vi "ADC_Config_Page.vi"() -> ()   [LabVIEW 2026, in "Core.lvlib"]
uses:
  Core.lvlib
  INL_DNL_Config_Page.vi
  TypeDefs/Enum_ADC_Tests.ctl
panel:
  in  "ADC Device Test":T1
  # "ADC Config Page"
  # "Instrument Specifications"
  # "Measurement Specifications"
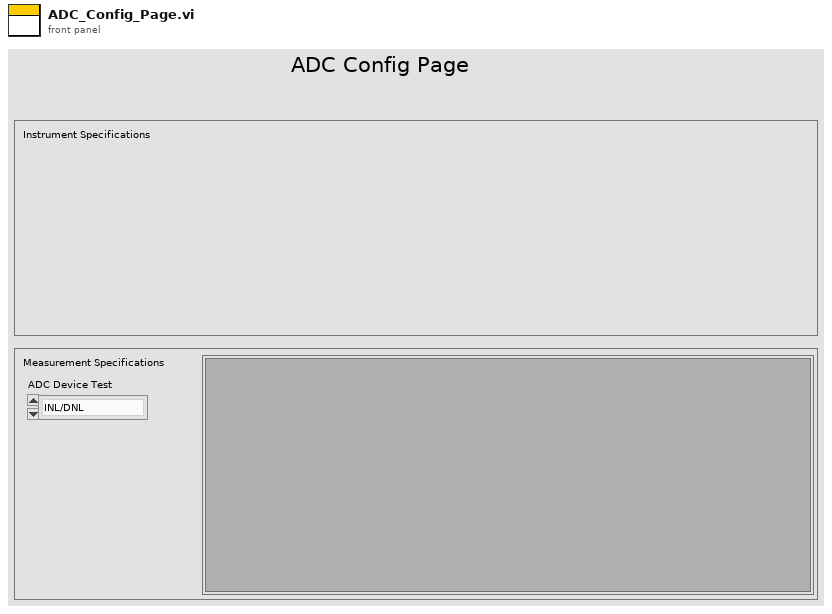
[diagram p1: front panel]
types:
  T1 = typedef "Core.lvlib/Enum_ADC_Tests.ctl" = enum16{"INL/DNL"}
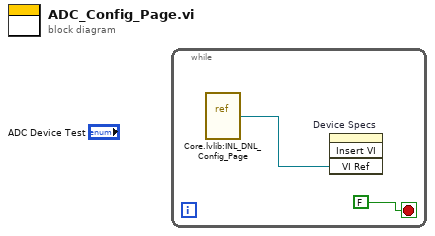
[diagram p0: block diagram]
diagram:
  n1 = while {
    stop <- FALSE stop-if-true
    n2 = vi-ref "Core.lvlib:INL_DNL_Config_Page.vi"() -> (w1:refnum<vi>)
    n3 = invoke on="Device Specs" class="SubPnl" method="Insert VI"("VI Ref"=w1) -> ()  [unwired: 3 in, 4 out]
  }
